vi "System Definition To Ports.vi"(8 "error in":errorcluster, 11 "custom device ref":T1 format="%.0x") -> (0 "error out":errorcluster, 2 "ports":T2[](array[typedef]), 3 "custom device ref out":T1 format="%.0x")   [LabVIEW 2020, in "AIM ARINC 429 Scripting.lvlib"]
uses:
  AIM ARINC 429 Scripting.lvlib
  Shared/Transfer Type.ctl
  <vilib>/NI/NI VeriStand Encoding and Decoding/Encoding.ctl
  <vilib>/NI/NI VeriStand Encoding and Decoding/Encoding and Decoding.lvlib
  Shared/Parameter Definition.ctl
  Shared/Direction.ctl
  Shared/VS Channel Definition for Parameter.ctl
  Shared/VS Channels Definition for Label.ctl
  Shared/VS Channels Definition for All Labels on Hardware Channel.ctl
  Shared/Transfer Speed.ctl
  <vilib>/NI VeriStand/Custom Device API/Custom Device Item Ref.ctl
  <vilib>/NI VeriStand/Custom Device API/Custom Device API.lvlib
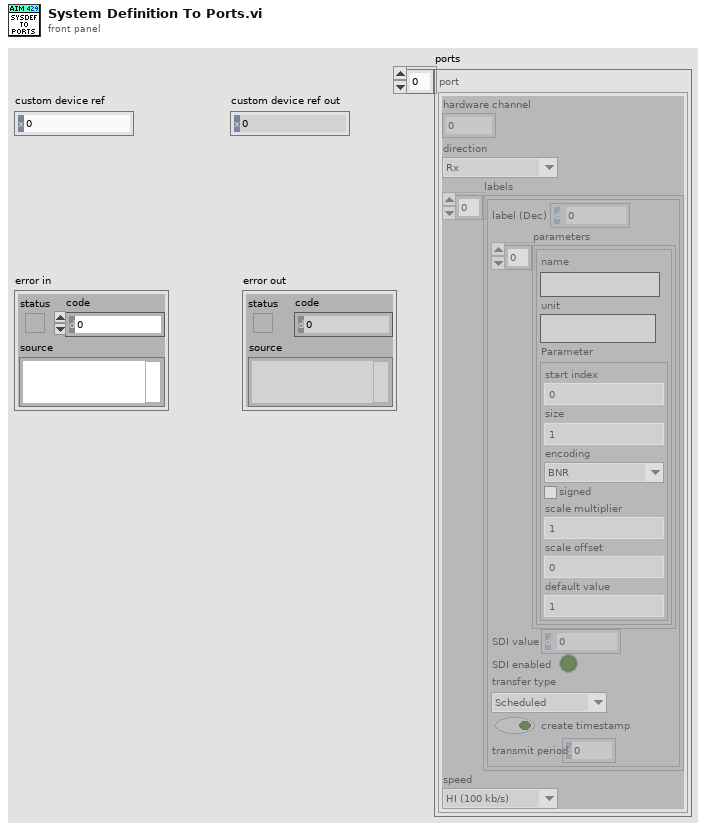
[diagram p1: front panel]
types:
  T1 = typedef "Custom Device API.lvlib/Custom Device Item Ref.ctl" = u64
  T2 = typedef "VS Channels Definition for All Labels on Hardware Channel.ctl" = cluster{"hardware channel":i32, "direction":T3, "labels":T4[], "speed":T9}
  T3 = typedef "Direction.ctl" = enum16{"Rx", "Tx"}
  T4 = typedef "VS Channels Definition for Label.ctl" = cluster{"label (Dec)":u32, "parameters":T5[], "SDI value":u8, "SDI enabled":bool, "transfer type":T8, "create timestamp":bool, "transmit period":u32}
  T5 = typedef "VS Channel Definition for Parameter.ctl" = cluster{"name":string, "unit":string, "Parameter":T6}
  T6 = typedef "Parameter Definition.ctl" = cluster{"start index":i32, "size":i32, "encoding":T7, "signed":bool, "scale multiplier":dbl, "scale offset":dbl, "default value":dbl}
  T7 = typedef "Encoding and Decoding.lvlib/Encoding.ctl" = enum16{"BNR", "BCD", "Discrete"}
  T8 = typedef "Transfer Type.ctl" = enum16{"Scheduled", "Acyclic", "Block", "Strobe"}
  T9 = typedef "Transfer Speed.ctl" = enum16{"LO (12.5 kb/s)", "HI (100 kb/s)"}
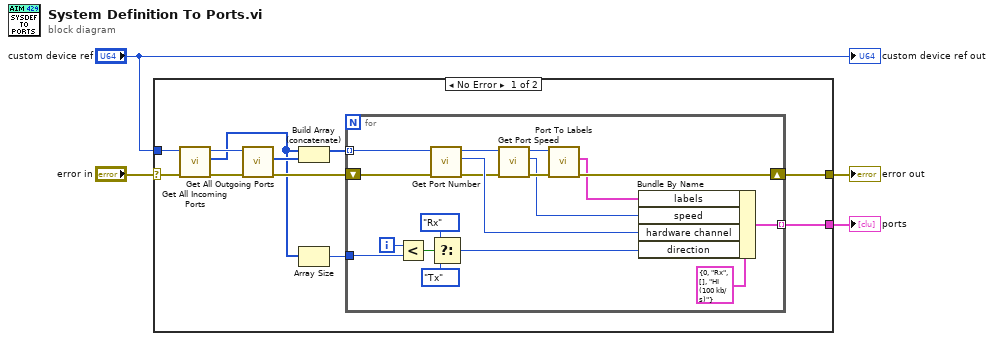
[diagram p0: block diagram]
diagram:
  n1 = case shown="No Error" "error in" {
    selector: "error in" -> [w14 w34]
    tunnel: "custom device ref" -> [w15 _]
    tunnel: [w7 w34] -> w4
    tunnel: [w8 _] -> w1
    frame No Error {
      n2 = call "Get All Incoming Ports.vi"("error in"=w14, "custom device ref"=w15) -> ("error out"=w13:errorcluster, "incoming ports"=w5:T1[], "custom device ref out"=w11:T1)  [unwired: 7 in]
      n3 = call "Get All Outgoing Ports.vi"("error in"=w13, "custom device ref"=w11) -> ("error out"=w9:errorcluster, "outgoing ports"=w12:T1[])  [unwired: 7 in, 1 out]
      n4 = Build Array (concatenate)(w5, w12) -> (w10:T1[])
      n5 = Array Size(array=w5) -> (size(s)=w6:i32)
      n6 = for {
        tunnel: w10 -> [w32] mode=indexing
        shift-right: [w23] -> w7
        shift-left: w9 -> [w33]
        tunnel: [w29] -> w8 mode=indexing
        tunnel: w6 -> [w24]
        i -> [w25]
        n7 = Less?(x=w25, y=w24) -> (x < y?=w26:bool)
        n8 = call "Get Port Number.vi"("error in"=w33, "port ref"=w32) -> ("error out"=w18:errorcluster, "port number"=w30:u16, "port ref out"=w19:T1)  [unwired: 6 in, 1 out]
        n9 = Select(t=Direction."Rx" ("direction"), s=w26, f=Direction."Tx" ("direction")) -> (s? t:f=w22:T3)
        n10 = call "Get Port Speed.vi"("error in"=w18, "port ref"=w19) -> ("error out"=w21:errorcluster, "speed"=w16:T9, "port ref out"=w20:T1)  [unwired: 7 in]
        n11 = call "Port To Labels.vi"("error in"=w21, "port ref"=w20) -> ("error out"=w23:errorcluster, "labels"=w17:T4[])  [unwired: 7 in, 1 out]
        n12 = Bundle By Name(cluster=T2 {"hardware channel"=0, "direction"=enum."Rx", "labels"=[], "speed"=enum."HI (100 kb/s)"} ("port"), "labels"=w17, "speed"=w16, "hardware channel"=w30, "direction"=w22) -> (w29:T2)
      }
    }
    frame Error {
    }
  }
  "error out" <- w4
  "ports" <- w1
  "custom device ref out" <- "custom device ref"
